vi "xnet_canopen_read_od.vi"(8 "error in (no error)":errorcluster, 10 "OD Index":T1 {"SubIndex" format="%.0x"; "Index" format="%.0x"}, 11 "xnet_co_handle_in":u64) -> (0 "error out":errorcluster, 2 "Value Bytes":u8[](array[numeric]), 3 "xnet_co_handle":u64)   [LabVIEW 2023, in "xnet_canopen.lvlib"]
uses:
  OD Batch/OD Batch.lvclass/OD Batch.ctl
  <vilib>/Utility/error.llb/Error Cluster From Error Code.vi
  xnet_canopen.lvlib
  typedef/od index.ctl
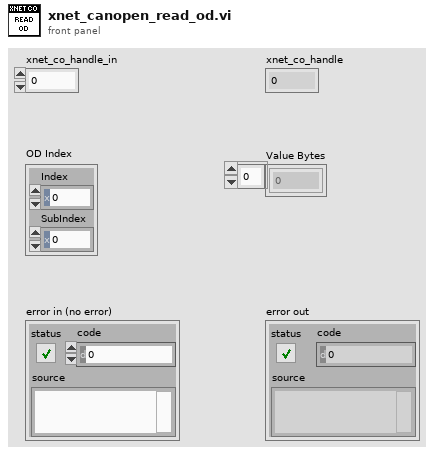
[diagram p1: front panel]
types:
  T1 = typedef "xnet_canopen.lvlib/od index.ctl" = cluster{"Index":u16, "SubIndex":u8}
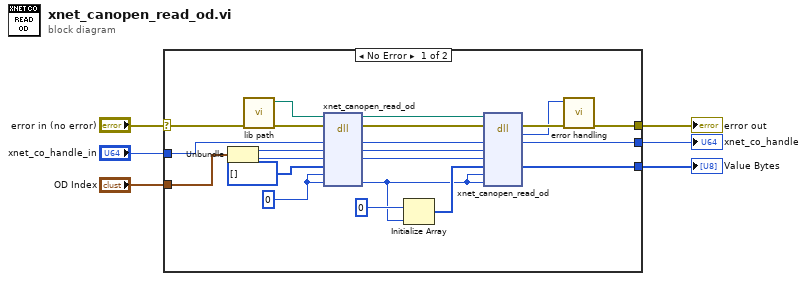
[diagram p0: block diagram]
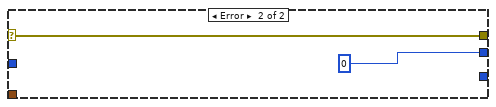
[diagram p2: hidden frame]
diagram:
  n1 = case shown="No Error" "error in (no error)" {
    selector: "error in (no error)" -> [w25 w29]
    tunnel: [w24 w29] -> w5
    tunnel: [w16 u64 0 ("phandle")] -> w4
    tunnel: "xnet_co_handle_in" -> [w26 _]
    tunnel: "OD Index" -> [w23 _]
    tunnel: [w7 _] -> w1
    frame No Error {
      w11 = u32 0 ("bufsize")
      n2 = Unbundle(w23) -> ("Index"=w22:u16, "SubIndex"=w21:u8)
      n3 = call "lib path.vi"() -> ("lib path"=w27:path)  [unwired: 11 in]
      n4 = dll-call lib="?" fn="xnet_canopen_read_od"(path in=w27, error in=w25, "handle"=w26, "index"=w22, "subindex"=w21, "buffer"=u8[] [], "bufsize"=w11, "expect_size"=w11) -> (path out=w14:path, error out=w19:errorcluster, "handle"=w15:u64, "index"=w13:u16, "subindex"=w12:u8, "expect_size"=w8:u32)  [unwired: 4 in]
      n5 = Initialize Array(u8 0 ("element"), w8) -> (w9:u8[])
      n6 = dll-call lib="?" fn="xnet_canopen_read_od"(path in=w14, error in=w19, "handle"=w15, "index"=w13, "subindex"=w12, "buffer"=w9, "bufsize"=w8, "expect_size"=w8) -> (error out=w18:errorcluster, "return type"=w17:i32, "handle"=w16:u64, "buffer"=w7:u8[])  [unwired: 5 in, 1 out]
      n7 = call "error handling.vi"("error in (no error)"=w18, "return val"=w17) -> ("error out"=w24:errorcluster)  [unwired: 9 in]
    }
    frame Error {
    }
  }
  "error out" <- w5
  "xnet_co_handle" <- w4
  "Value Bytes" <- w1
